vi "GetTestTypeDescv3NoRbac.vi"() -> ()   [LabVIEW 2017]
uses:
  <vilib>/httpClient/LabVIEWHTTPClient.lvlib
  <vilib>/Analysis/NI_AALBase.lvlib
panel:
  out "test_property":T1
  out "standard deviation":dbl format="%0.2f"
  out "mean":dbl format="%0.2f"
  out "error out":errorcluster
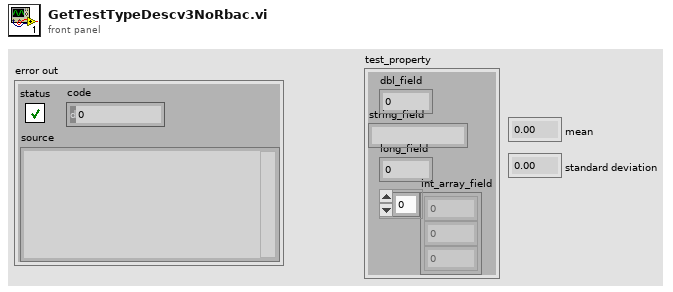
[diagram p1: front panel]
types:
  T1 = cluster{"dbl_field":dbl, "string_field":string, "long_field":i64, "int_array_field":i32[]}
  T2 = typedef "LabVIEWHTTPClient.lvlib/ClientHandle.ctl" = refnum<k1>
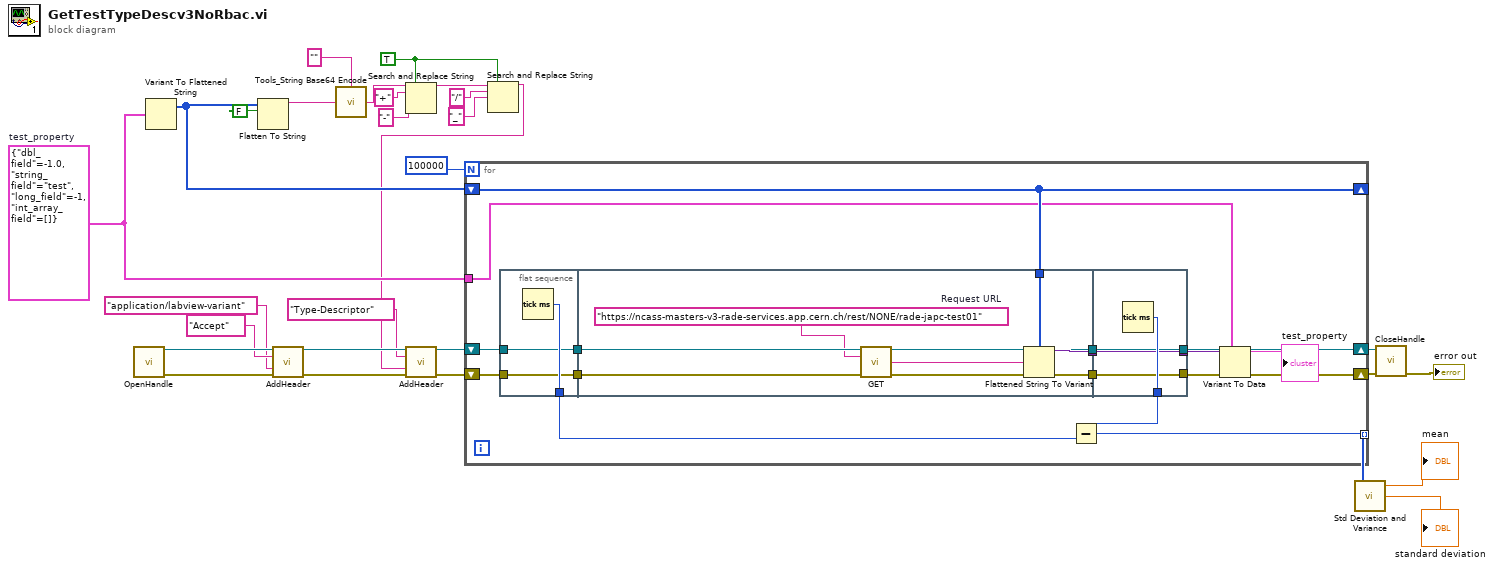
[diagram p0: block diagram]
diagram:
  w5 = TRUE ("replace all? (F)")
  w10 = T1 {"dbl_field"=-1.0, "string_field"="test", "long_field"=-1, "int_array_field"=[]}  # test_property
  n1 = call <vilib>:"OpenHandle.vi"() -> ("client handle out"=w25:T2, "error out"=w26:errorcluster)  [unwired: 14 in]
  n2 = Variant To Flattened String(Variant=w10) -> (1:w18:i16[])  [unwired: 1 out]
  n3 = Flatten To String(anything=w18, prepend array or string size? (T)=FALSE) -> (data string=w24:string)  [unwired: 2 in, 2 out]
  n4 = call <vilib>:"AddHeader.vi"("client handle"=w25, "header"="Accept", "value"="application/labview-variant", "error in (no error)"=w26) -> ("client handle out"=w27:T2, "error out"=w28:errorcluster)  [unwired: 10 in]
  n5 = call <userlib>:"Tools_String Base64 Encode.vi"("Normal String"=w24, "Line separator (\\n)"="") -> ("Base64 String"=w7:string)
  n6 = Search and Replace String(replace all?=w5, input string=w7, search string="+" ("substring (\"\")"), replace string="-" ("replace string (\"\")")) -> (result string=w6:string)  [unwired: 4 in, 3 out]
  n7 = Search and Replace String(replace all?=w5, input string=w6, search string="/" ("substring (\"\")"), replace string="_" ("replace string (\"\")")) -> (result string=w2:string)  [unwired: 4 in, 3 out]
  n8 = call <vilib>:"AddHeader.vi"("client handle"=w27, "header"="Type-Descriptor", "value"=w2, "error in (no error)"=w28) -> ("client handle out"=w11:T2, "error out"=w19:errorcluster)  [unwired: 10 in]
  n9 = for {
    N: 100000 -> [_]
    shift-right: [w46] -> _
    shift-left: w18 -> [w46]
    tunnel: w10 -> [w41]
    tunnel: [w37] -> w14 mode=indexing
    shift-right: [w39] -> w16
    shift-left: w11 -> [w35]
    shift-right: [w30] -> w15
    shift-left: w19 -> [w33]
    n10 = flat-sequence {
      tunnel: [w49] -> w45
      tunnel: [w48] -> w36
      tunnel: w35 -> [w48]
      tunnel: [w47] -> w34
      tunnel: w33 -> [w47]
      tunnel: w46 -> [w57]
      tunnel: [w56] -> w43
      tunnel: [w55] -> w40
      tunnel: [w51] -> w38
      tunnel: w36 -> [w54]
      tunnel: w34 -> [w53]
      tunnel: [w62] -> w44
      tunnel: w43 -> [w61]
      tunnel: [w61] -> w42
      tunnel: [w60] -> w39
      tunnel: w40 -> [w60]
      tunnel: [w59] -> w31
      tunnel: w38 -> [w59]
      frame #0 {
        n11 = Tick Count (ms)() -> (millisecond timer value=w49:u32)
      }
      frame #1 {
        w50 = "https://ncass-masters-v3-rade-services.app.cern.ch/rest/NONE/rade-japc-test01"  # Request URL
        n12 = call <vilib>:"GET.vi"("client handle"=w54, "url"=w50, "error in (no error)"=w53) -> ("client handle out"=w55:T2, "body"=w58:string, "error out"=w52:errorcluster)  [unwired: 9 in, 1 out]
        n13 = Flattened String To Variant(4:w52, 6:w58, 7:w57) -> (0:w51:errorcluster, 3:w56:variant)
      }
      frame #2 {
        n14 = Tick Count (ms)() -> (millisecond timer value=w62:u32)
      }
    }
    n15 = Subtract(x=w44, y=w45) -> (x-y=w37:u32)
    n16 = Variant To Data(error in=w31, type=w41, Variant=w42) -> (data=→"test_property":T1, error out=w30:errorcluster)
  }
  n17 = call <vilib>:"Std Deviation and Variance.vi"("X"=w14) -> ("mean"=→"mean":dbl, "standard deviation"=→"standard deviation":dbl)  [unwired: 1 in, 1 out]
  n18 = call <vilib>:"CloseHandle.vi"("client handle"=w16, "error in (no error)"=w15) -> ("error out"=→"error out":errorcluster)  [unwired: 13 in]
